vi "HandleItemActivation.vi"(8 "error in (no error)":errorcluster, 11 "GettingStartedWindow.lvlib:Web.lvclass":refnum<class "Web.lvclass">) -> (0 "error out":errorcluster, 3 "GettingStartedWindow.lvlib:Web.lvclass 2":refnum<class "Web.lvclass">)   [LabVIEW 2023, in "GettingStartedWindow.lvlib" / "Web.lvclass"]
uses:
  <resource>/modes/FRC/GSW/Classes/Web/Web.lvclass
  <resource>/modes/FRC/GSW/Classes/Web/Web.lvclass/Web.ctl
  <vilib>/Platform/browser.llb/Open URL in Default Browser (string).vi
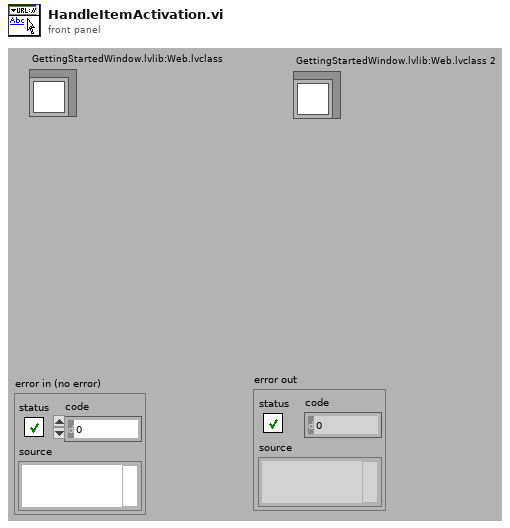
[diagram p1: front panel]
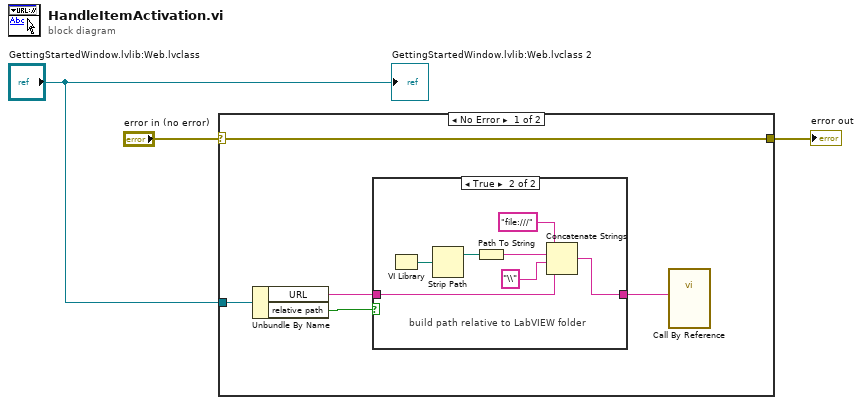
[diagram p0: block diagram]
diagram:
  n1 = case shown="No Error" "error in (no error)" {
    selector: "error in (no error)" -> [w8 w17]
    tunnel: [w8 w17] -> w2
    tunnel: "GettingStartedWindow.lvlib:Web.lvclass" -> [w7 _]
    frame No Error {
      n2 = Unbundle By Name(w7) -> ("URL"=w5:string, "relative path"=w6:bool)
      n3 = case shown="True" w6 {
        tunnel: w5 -> [w9 w11]
        tunnel: [w9 w10] -> w4
        frame False {
        }
        frame True {
          # "build path relative to LabVIEW folder"
          n4 = VI Library() -> (path=w12:path)
          n5 = Strip Path(path=w12) -> (stripped path=w13:path)  [unwired: 1 out]
          n6 = Path To String(path=w13) -> (string=w14:string)
          n7 = Concatenate Strings("file:///" ("string"), w14, "\\", w11) -> (w10:string)
        }
      }
      n8 = call-by-ref "?"("URL"=w4) -> ()  [unwired: 3 in, 8 out]
    }
    frame Error {
    }
  }
  "error out" <- w2
  "GettingStartedWindow.lvlib:Web.lvclass 2" <- "GettingStartedWindow.lvlib:Web.lvclass"
